vi "FuncVI-QueueLength.vi"(5 "InstanceRef":T2, 9 "arg list":T1[](array[typedef]) {"num" format="%.2f"}) -> (0 "error out":bool, 3 "result":T1 {"num" format="%.2f"})   [LabVIEW 2021]
doc: "::: CalcExpress Toolkit :::\nCopyright (c) 2000-2026 Konstantin Shifershteyn. All rights reserved."
uses:
  cetypes.llb/CalcExpress Function Argument Info.ctl
  cetypes.llb/CalcExpress Instance RefNum.ctl
panel:
  in  "max arg num":i32=1
  in  "min arg num":i32=1
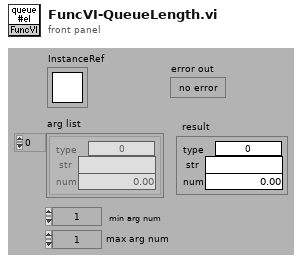
[diagram p1: front panel]
types:
  T1 = typedef "CalcExpress Function Argument Info.ctl" = cluster{"type":u32, "str":string, "num":dbl}
  T2 = typedef "CalcExpress Instance RefNum.ctl" = refnum<k1>
  T3 = enum32{"String", "DBL Number", "identifier", "1D Array of DBL", "2D Array of DBL", "CDB Number", "1D Array of CDB", "2D Array of CDB", "1D Array of String", "2D Array of String", "Unknown data type"}
  T4 = cluster{"data type":enum32{"String", "DBL Number", "identifier", "1D Array of DBL", "2D Array of DBL", "CDB Number", "1D Array of CDB", "2D Array of CDB", "1D Array of String", "2D Array of String", "Unknown data type"}, string, dbl}
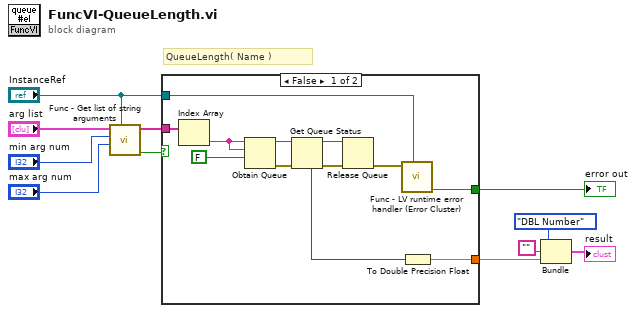
[diagram p0: block diagram]
diagram:
  # "QueueLength( Name )"
  n1 = call "Func - Get list of string arguments.vi"("InstanceRef"="InstanceRef", "max arg num"="max arg num", "min arg num"="min arg num", "arg list"="arg list") -> ("error out"=w4:bool, "val list"=w10:string[])  [unwired: 4 in]
  n2 = case shown="False" w4 {
    selector: w4 -> [_ w24]
    tunnel: w10 -> [w23 _]
    tunnel: "InstanceRef" -> [w21 _]
    tunnel: [w22 _] -> w5
    tunnel: [w20 w24] -> w3
    frame False {
      n3 = Index Array(array=w23) -> (element=w19:string)  [unwired: 1 in]
      n4 = Obtain Queue(name (unnamed)=w19, element data type=w19, create if not found? (T)=FALSE) -> (queue out=w16:refnum<queue>, error out=w17:errorcluster)  [unwired: 2 in, 1 out]
      n5 = Get Queue Status(queue=w16, error in (no error)=w17) -> (queue out=w15:refnum<queue>, error out=w14:errorcluster, # elements in queue=w12:i32)  [unwired: 1 in, 5 out]
      n6 = Release Queue(queue=w15, error in (no error)=w14) -> (error out=w13:errorcluster)  [unwired: 1 in, 2 out]
      n7 = call "Func - LV runtime error handler (Error Cluster).vi"("InstanceRef"=w21, "LabVIEW error"=w13) -> ("error out"=w20:bool)  [unwired: 4 in, 3 out]
      n8 = To Double Precision Float(number=w12) -> (double precision float=w22:dbl)
    }
    frame True {
    }
  }
  "error out" <- w3
  n9 = Bundle("data type"=T3."DBL Number", "", w5) -> (→"result":T4)  [unwired: 1 in]
